vi "Temp Coef to Color Converter.vi"(2 "Temp Coef select":T1=enum."Red - 50 ppm/K") -> (6 "Temp Coef Color":u32(colorbox))   [LabVIEW 2018, in "Resistance Colors.lvlib"]
doc: "Converts the selected Temperature Coefficient Enum value into the corresponding color for the resistor band.\n\nThe VI receives the <b>Temp Coef select</b> input and returns the corresponding resistor band color through <b>Temp Coef Color</b>.\n\nThe color is determined by mapping the selected Enum item to the corresponding color constant."
uses:
  Resistance Colors.lvlib
  Resistor Controls/Temp Coefficient--enum.ctl
  Band Colors/Band Colors.lvlib
  Resistor Controls/Resistance Controls.lvlib
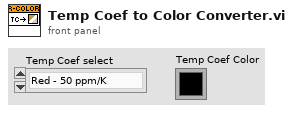
[diagram p1: front panel]
types:
  T1 = typedef "Resistance Controls.lvlib/Temp Coefficient--enum.ctl" = enum16{"Grey - 1 ppm/K", "Violet - 5 ppm/K", "Blue - 10 ppm/K", "Green - 20 ppm/K", "Yellow - 25 ppm/K", "Orange - 15 ppm/K", "Red - 50 ppm/K", "Brown - 100 ppm/K", "Black - 250 ppm/K"}
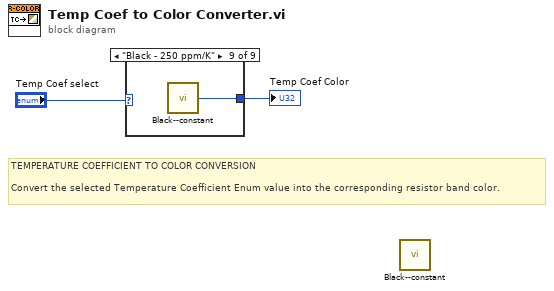
[diagram p0: block diagram]
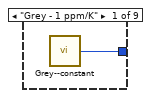
[diagram p2: hidden frame]
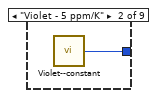
[diagram p3: hidden frame]
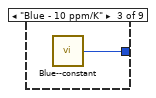
[diagram p4: hidden frame]
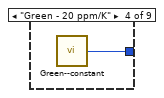
[diagram p5: hidden frame]
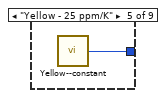
[diagram p6: hidden frame]
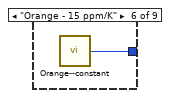
[diagram p7: hidden frame]
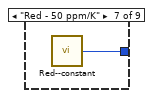
[diagram p8: hidden frame]
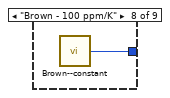
[diagram p9: hidden frame]
diagram:
  # "TEMPERATURE COEFFICIENT TO COLOR CONVERSION\n\nConvert the selected Temperature Coefficient Enum value into the corresponding resistor band color."
  n1 = case shown="\"Black - 250 ppm/K\"" "Temp Coef select" {
    tunnel: [w3 w4 w5 w6 w7 w8 w9 w10 w11] -> w1
    frame "Grey - 1 ppm/K" {
      n2 = call "Grey--constant.vi"() -> ("Gray"=w3:u32)  [unwired: 5 in]
    }
    frame "Violet - 5 ppm/K" {
      n3 = call "Violet--constant.vi"() -> ("Violet"=w4:u32)  [unwired: 5 in]
    }
    frame "Blue - 10 ppm/K" {
      n4 = call "Blue--constant.vi"() -> ("Blue"=w5:u32)  [unwired: 5 in]
    }
    frame "Green - 20 ppm/K" {
      n5 = call "Green--constant.vi"() -> ("Green"=w6:u32)  [unwired: 5 in]
    }
    frame "Yellow - 25 ppm/K" {
      n6 = call "Yellow--constant.vi"() -> ("Yellow"=w7:u32)  [unwired: 5 in]
    }
    frame "Orange - 15 ppm/K" {
      n7 = call "Orange--constant.vi"() -> ("Orange"=w8:u32)  [unwired: 5 in]
    }
    frame "Red - 50 ppm/K" {
      n8 = call "Red--constant.vi"() -> ("Red"=w9:u32)  [unwired: 5 in]
    }
    frame "Brown - 100 ppm/K" {
      n9 = call "Brown--constant.vi"() -> ("Brown"=w10:u32)  [unwired: 5 in]
    }
    frame "Black - 250 ppm/K" {
      n10 = call "Black--constant.vi"() -> ("Black"=w11:u32)  [unwired: 5 in]
    }
  }
  "Temp Coef Color" <- w1
  n11 = call "Black--constant.vi"() -> ()  [unwired: 5 in, 1 out]
